vi "Power Clear Request.vi"(8 "error in (no error)":errorcluster, 10 "Power Request Type":T1, 11 "Handle in":i64) -> (0 "error out":errorcluster, 2 "Success?":bool, 3 "Handle out":i64)   [LabVIEW 2024, in "Power Requests.lvlib"]
uses:
  Power Requests.lvlib
  Type Defs/Power Request Type.ctl
  kernel32.dll
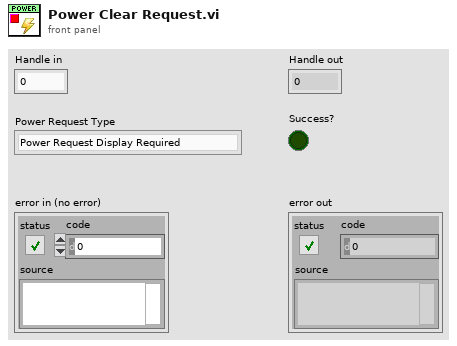
[diagram p1: front panel]
types:
  T1 = typedef "Power Requests.lvlib/Power Request Type.ctl" = enum32{"Power Request Display Required", "Power Request System Required", "Power Request Away Mode Required", "Power Request Execution Required"}
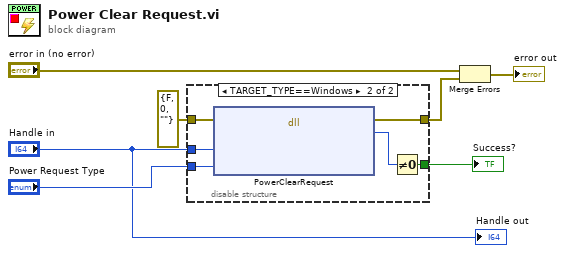
[diagram p0: block diagram]
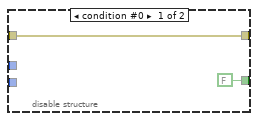
[diagram p2: hidden frame]
diagram:
  n1 = disable-structure shown="TARGET_TYPE==Windows" {
    disable-tunnel: [w9 w15] -> w3
    disable-tunnel: errorcluster {"status"=FALSE, "code"=0, "source"=""} ("error in (no error)") -> [w9 w14]
    disable-tunnel: "Handle in" -> [_ w13]
    disable-tunnel: "Power Request Type" -> [_ w12]
    disable-tunnel: [FALSE w10] -> w5
    frame condition #0 {
    }
    frame condition #1 (active) {
      n2 = dll-call lib="kernel32.dll" fn="PowerClearRequest"(error in=w14, "_In_ HANDLE"=w13, "_In_ POWER_REQUEST_TYPE"=w12) -> (error out=w15:errorcluster, "BOOL"=w11:i32)  [unwired: 4 in, 1 out]
      n3 = Not Equal To 0?(x=w11) -> (x != 0?=w10:bool)
    }
  }
  "Success?" <- w5
  n4 = Merge Errors("error in (no error)", w3) -> (→"error out":errorcluster)
  "Handle out" <- "Handle in"
